vi "Demo UNO Q - blink.vi"() -> ()   [LabVIEW 2021]
uses:
  <vilib>/httpClient/ClientHandle.ctl
  <vilib>/httpClient/POSTBuffer.vi
  <vilib>/httpClient/LabVIEWHTTPClient.lvlib
panel:
  out "error out":errorcluster
  out "body":string
  out "headers":string
  out "Boolean":bool
  in  "stop":bool
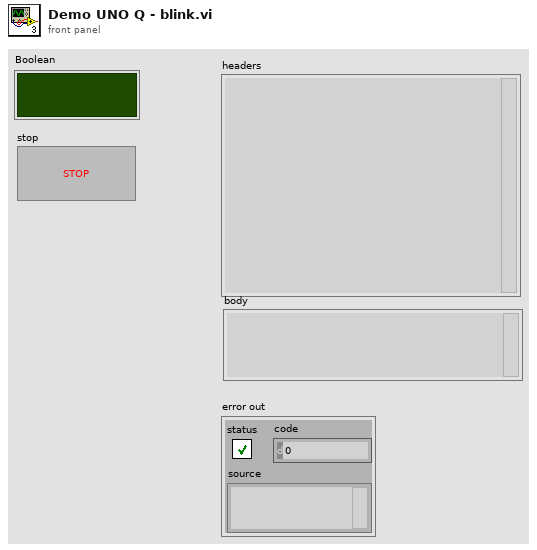
[diagram p1: front panel]
types:
  T1 = typedef "UNOQ Session.ctl" = cluster{"HTTP client":T2, "Base URL":string, "Connected":bool}
  T2 = typedef "LabVIEWHTTPClient.lvlib/ClientHandle.ctl" = refnum<k1>
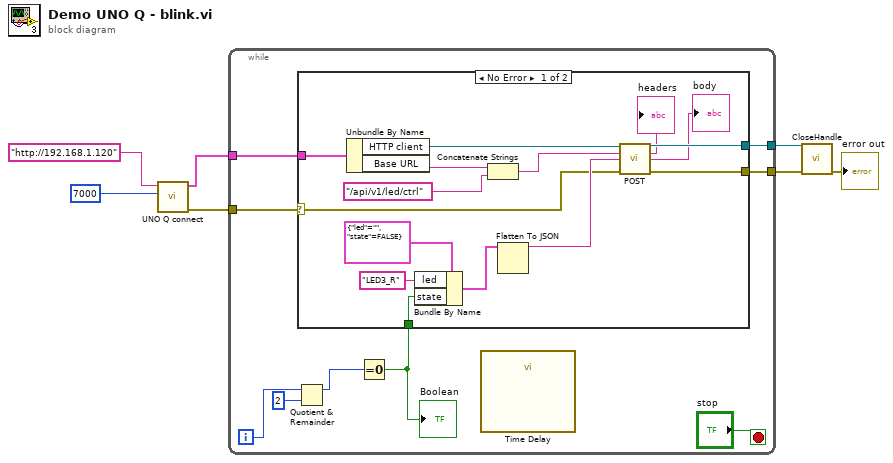
[diagram p0: block diagram]
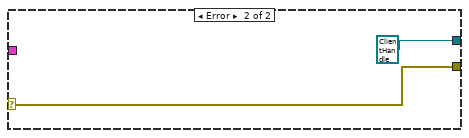
[diagram p2: hidden frame]
diagram:
  n1 = call "UNO Q connect.vi"("port"=u32 7000, "Base URL"="http://192.168.1.120") -> ("error out"=w5:errorcluster, "Session out"=w4:T1)  [unwired: 4 in]
  n2 = while {
    tunnel: w5 -> [w16]
    tunnel: w4 -> [w15]
    tunnel: [w14] -> w3
    tunnel: [w9] -> w2
    i -> [w12]
    stop <- "stop" stop-if-true
    n3 = Quotient & Remainder(x=w12, y=2) -> (x-y*floor(x/y)=w10:i32)  [unwired: 1 out]
    n4 = Equal To 0?(x=w10) -> (x = 0?=w8:bool)
    "Boolean" <- w8
    n5 = case shown="No Error" w16 {
      selector: w16 -> [w20 w32]
      tunnel: w15 -> [w28 _]
      tunnel: [w24 T2 refnum ("client handle out")] -> w14
      tunnel: w8 -> [w23 _]
      tunnel: [w19 w32] -> w9
      frame No Error {
        n6 = Unbundle By Name(w28) -> ("HTTP client"=w30:T2, "Base URL"=w31:string)
        n7 = Bundle By Name(cluster=cluster{"led":string, "state":bool} {"led"="", "state"=FALSE}, "led"="LED3_R", "state"=w23) -> (w22:cluster{"led":string, "state":bool})
        n8 = Concatenate Strings(w31, "/api/v1/led/ctrl" ("string")) -> (w27:string)
        n9 = Flatten To JSON(anything=w22) -> (JSON string=w21:string)  [unwired: 2 in, 1 out]
        n10 = call-poly <vilib>:"POST.vi"("client handle"=w30, "url"=w27, "buffer"=w21, "error in (no error)"=w20) -> ("client handle out"=w24:T2, "headers"=→"headers":string, "body"=→"body":string, "error out"=w19:errorcluster)  [unwired: 8 in]
      }
      frame Error {
      }
    }
    n11 = call "Time Delay"() -> ()  [unwired: 11 in, 1 out]
  }
  n12 = call <vilib>:"CloseHandle.vi"("client handle"=w3, "error in (no error)"=w2) -> ("error out"=→"error out":errorcluster)  [unwired: 13 in]
